vi "Scripting_ChangeBaseClassInSubClass.vi"(0 "SubClass":refnum<vi>, 1 "NewBaseClass":path=path "C:/Projects/Base2_class/Base2.lvclass", 2 "GOOP4Style":bool, 5 "error in (no error)":errorcluster) -> (19 "error out":errorcluster={"status"=TRUE, "code"=1055, "source"="Property Node in Scripting_ConvertBaseClassToSubClass.vi"})   [LabVIEW 2020]
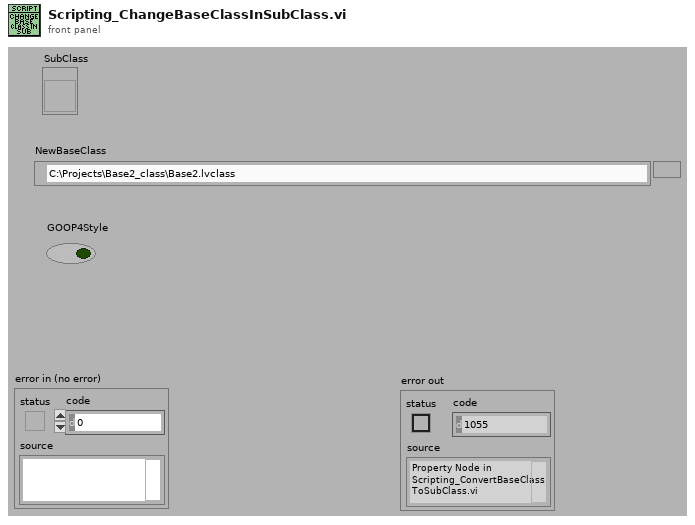
[diagram p1: front panel]
types:
  T1 = cluster{"NewBaseClass":refnum<vi>, "NewBaseClassPath":path, "SubClass":refnum<vi>, "NewBaseClassName":string, "AllBaseClassFiles":path[], "ClassVIs":refnum<vi>[], "CurrentBaseClassRef":refnum<vi>, "CurrentBaseClassPath":path, "CurrentRootBaseClassPath":path, "NewRootBaseClassPath":path}
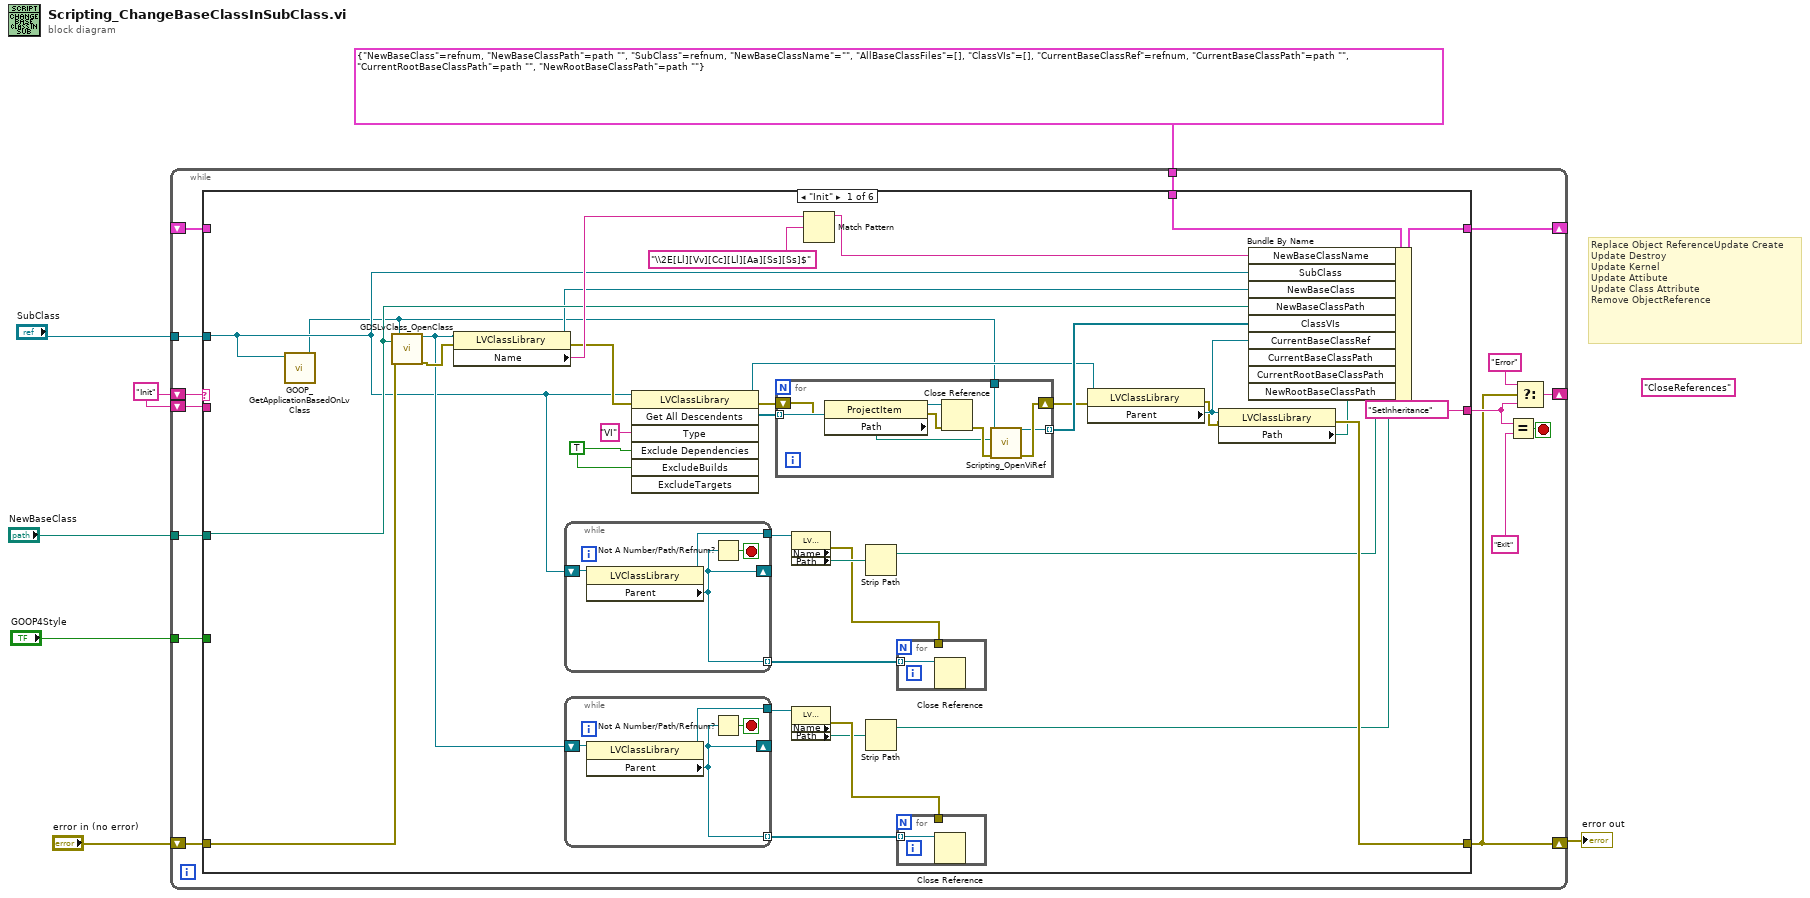
[diagram p0: block diagram]
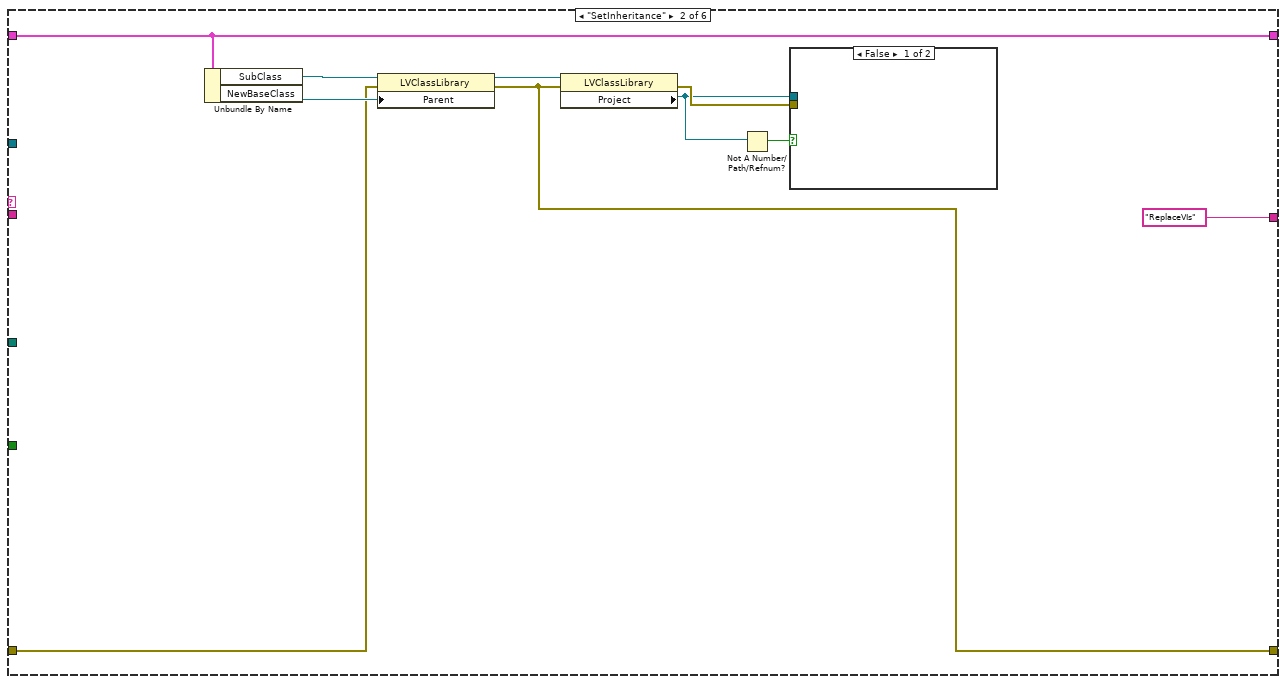
[diagram p2: hidden frame]
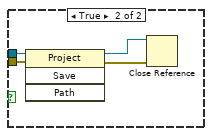
[diagram p3: hidden frame]
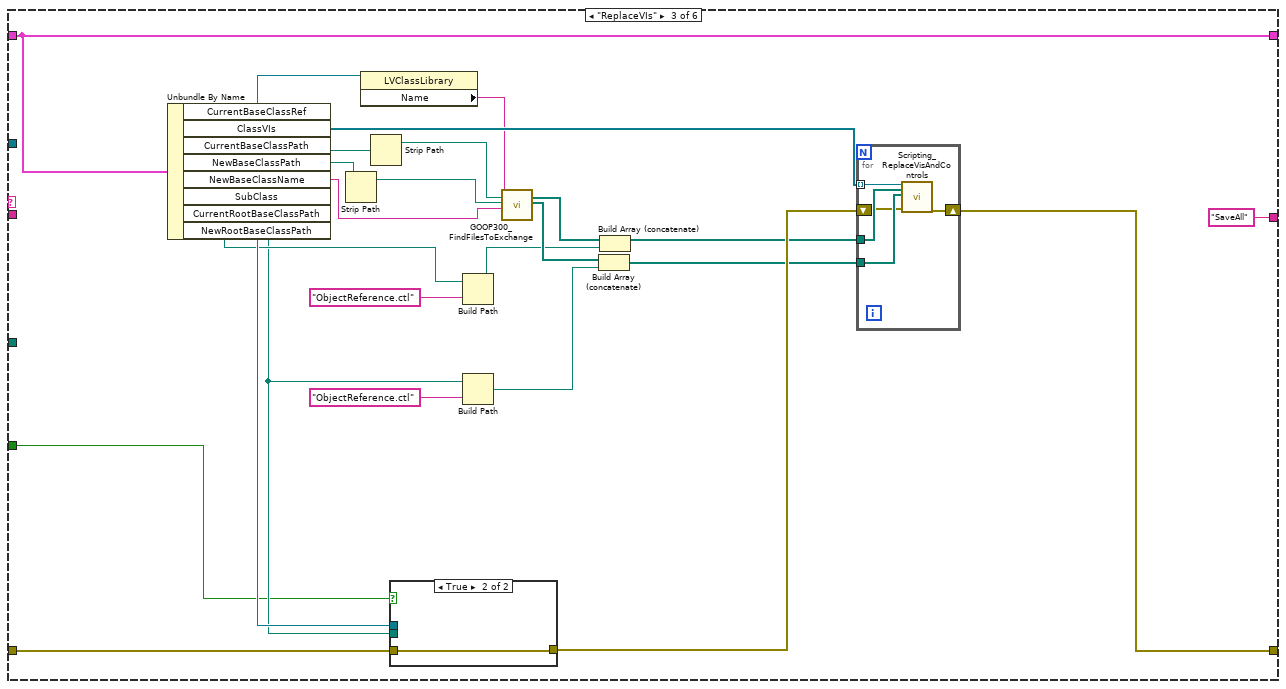
[diagram p4: hidden frame]
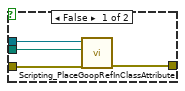
[diagram p5: hidden frame]
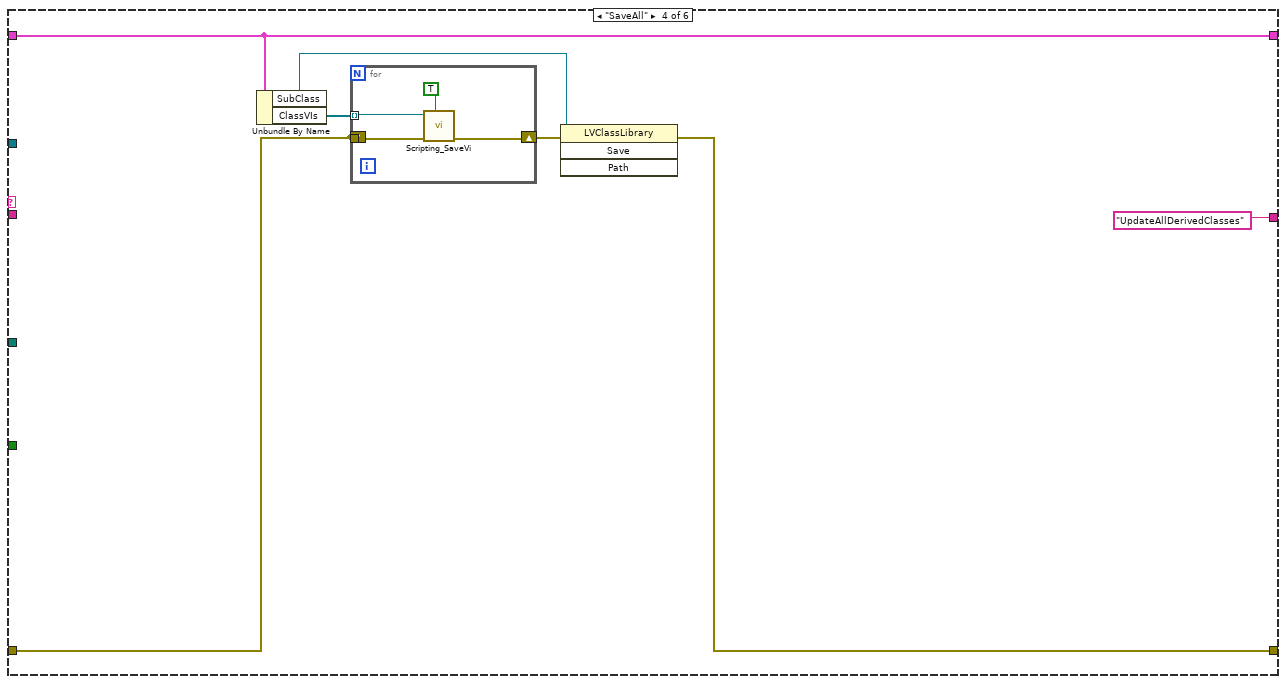
[diagram p6: hidden frame]
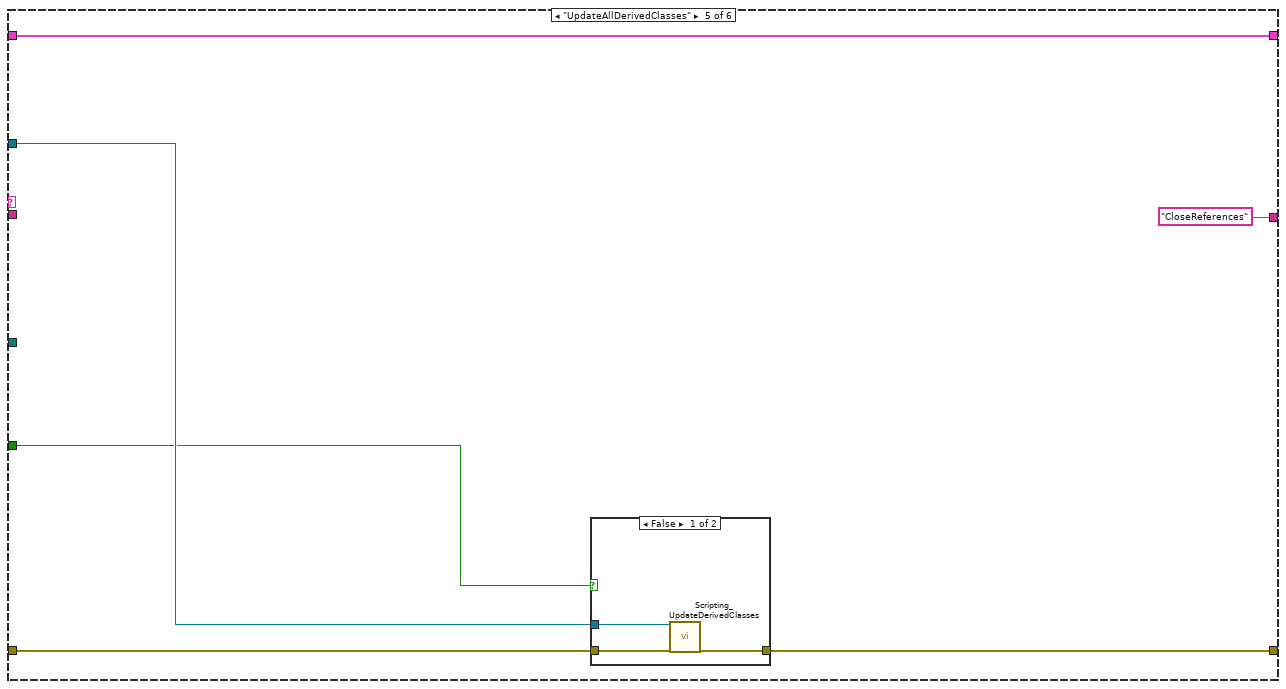
[diagram p7: hidden frame]
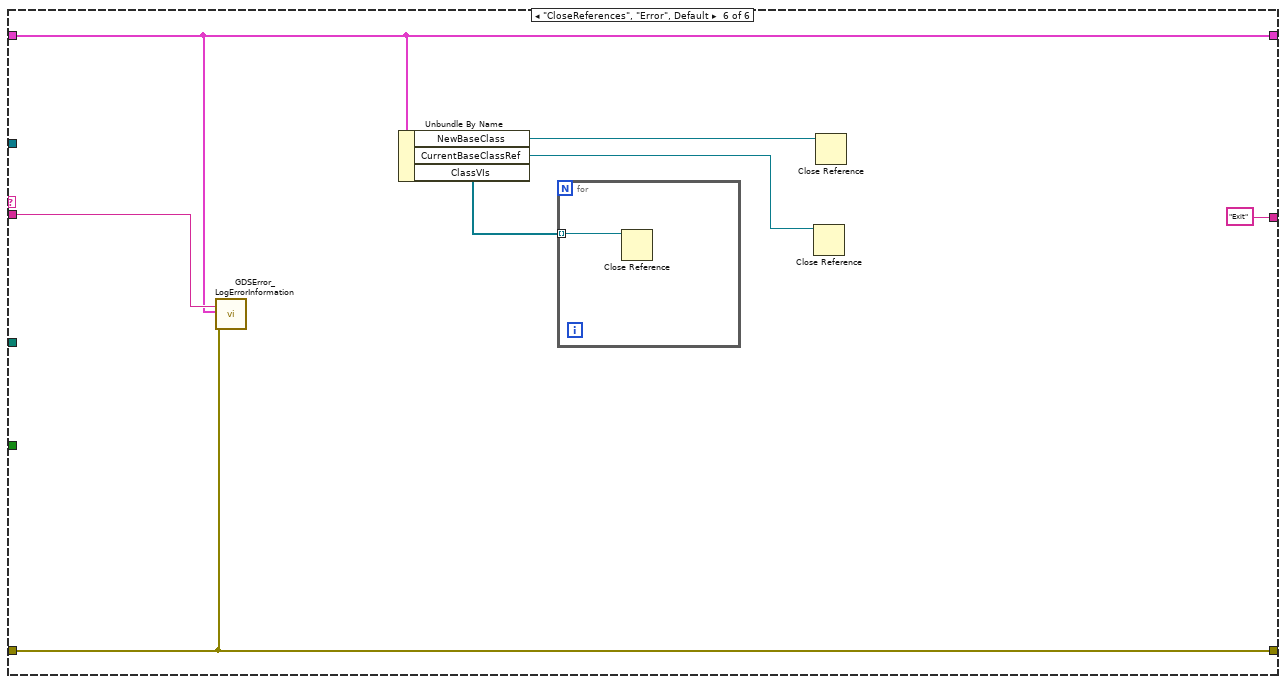
[diagram p9: hidden frame]
diagram:
  (unwired) "CloseReferences"
  w2 = "Init"
  # "Replace Object ReferenceUpdate Create\nUpdate Destroy\nUpdate Kernel\nUpdate Attibute\nUpdate Class Attribute\nRemove ObjectReference"
  n1 = while {
    shift-right: [w15] -> w6
    shift-left: "error in (no error)" -> [w22]
    shift-right: [w20] -> _
    shift-left: w2 -> [w21]
    shift-right: [w14] -> _
    shift-left: _ -> [w13]
    tunnel: "SubClass" -> [w12]
    tunnel: T1 {"NewBaseClass"=refnum, "NewBaseClassPath"=path "", "SubClass"=refnum, "NewBaseClassName"="", "AllBaseClassFiles"=[], "ClassVIs"=[], "CurrentBaseClassRef"=refnum, "CurrentBaseClassPath"=path "", "CurrentRootBaseClassPath"=path "", "NewRootBaseClassPath"=path ""} -> [w11]
    tunnel: "NewBaseClass" -> [w10]
    shift-left: w2 -> [w9]
    tunnel: "GOOP4Style" -> [w8]
    stop <- w19 stop-if-true
    n2 = case shown="\"Init\"" w21 {
      tunnel: w22 -> [w39 w83 w106 w130 w140 w149]
      tunnel: [w47 w77 w114 w127 w138 w149] -> w15
      tunnel: ["SetInheritance" "ReplaceVIs" "SaveAll" "UpdateAllDerivedClasses" "CloseReferences" "Exit"] -> w16
      tunnel: [w57 w85 w110 w131 w141 w147] -> w14
      tunnel: w13 -> [_ w85 w110 w131 w141 w147]
      tunnel: w12 -> [w24 _ _ _ w139 _]
      tunnel: w11 -> [w54 _ _ _ _ _]
      tunnel: w10 -> [w44 _ _ _ _ _]
      tunnel: w9 -> [_ _ _ _ _ w148]
      tunnel: w8 -> [_ _ w91 _ w137 _]
      frame "Init" {
        w25 = TRUE ("ExcludeDependencies")
        n3 = call "GOOP_GetApplicationBasedOnLvClass.vi"("LVClassLibrary in"=w24) -> ("Application out"=w23:refnum<vi>)  [unwired: 9 in, 1 out]
        n4 = call "GDSLvClass_OpenClass.vi"("ClassToOpen"=w44, "error in (no error)"=w39, "Project/ApplicationRef(If empty, currect active project will be used)"=w23) -> ("LVClass.Open"=w27:refnum<vi>, "error out"=w40:errorcluster)  [unwired: 15 in]
        n5 = property class="LVClassLibrary"(reference=w27, error in=w40) -> (reference out=w37:refnum<vi>, error out=w38:errorcluster, "Name"=w52:string)
        n6 = while {
          shift-right: [w65] -> _
          shift-left: w24 -> [w66]
          tunnel: [w65] -> w36 mode=indexing
          tunnel: [w64] -> w35
          stop <- w67 stop-if-true
          n7 = property class="LVClassLibrary"(reference=w66) -> (reference out=w64:refnum<vi>, "Parent"=w65:refnum<vi>)  [unwired: 1 in, 1 out]
          n8 = Not A Number/Path/Refnum?(number/path/refnum=w65) -> (NaN/Path/Refnum?=w67:bool)
        }
        n9 = while {
          shift-right: [w60] -> _
          shift-left: w27 -> [w61]
          tunnel: [w60] -> w28 mode=indexing
          tunnel: [w59] -> w29
          stop <- w62 stop-if-true
          n10 = property class="LVClassLibrary"(reference=w61) -> (reference out=w59:refnum<vi>, "Parent"=w60:refnum<vi>)  [unwired: 1 in, 1 out]
          n11 = Not A Number/Path/Refnum?(number/path/refnum=w60) -> (NaN/Path/Refnum?=w62:bool)
        }
        n12 = invoke class="LVClassLibrary" method="Get All Descendents"(reference=w24, error in=w38, "Type"="VI", "Exclude Dependencies"=w25, "ExcludeBuilds"=w25) -> (reference out=w43:refnum<vi>, error out=w55:errorcluster, "All Descendents"=w56:refnum<vi>[])  [unwired: 2 in, 4 out]
        n13 = for {
          tunnel: w56 -> [w76] mode=indexing
          shift-right: [w71] -> w48
          shift-left: w55 -> [w73]
          tunnel: [w69] -> w49 mode=indexing
          tunnel: w23 -> [w68]
          n14 = property class="ProjectItem"(reference=w76, error in=w73) -> (reference out=w75:refnum<vi>, error out=w74:errorcluster, "Path"=w70:path)
          n15 = Close Reference(reference=w75, error in (no error)=w74) -> (error out=w72:errorcluster)
          n16 = call "Scripting_OpenViRef.vi"("error in"=w72, "ViPath/ViName/Viref"=w70, "AppRef"=w68) -> ("error out"=w71:errorcluster, "vi reference"=w69:refnum<vi>)  [unwired: 6 in, 1 out]
        }
        n17 = property class="LVClassLibrary" props=["Name", "Path"](reference=w35) -> (error out=w33:errorcluster, "Path"=w34:path)  [unwired: 1 in, 2 out]
        n18 = property class="LVClassLibrary" props=["Name", "Path"](reference=w29) -> (error out=w31:errorcluster, "Path"=w30:path)  [unwired: 1 in, 2 out]
        n19 = Match Pattern(string=w52, regular expression="\\2E[Ll][Vv][Cc][Ll][Aa][Ss][Ss]$") -> (before substring=w51:string)  [unwired: 1 in, 3 out]
        n20 = Strip Path(path=w34) -> (stripped path=w32:path)  [unwired: 1 out]
        n21 = Strip Path(path=w30) -> (stripped path=w26:path)  [unwired: 1 out]
        n22 = for {
          tunnel: w36 -> [w63] mode=indexing
          tunnel: w33 -> [_]
          n23 = Close Reference(reference=w63) -> ()  [unwired: 1 in, 1 out]
        }
        n24 = for {
          tunnel: w28 -> [w58] mode=indexing
          tunnel: w31 -> [_]
          n25 = Close Reference(reference=w58) -> ()  [unwired: 1 in, 1 out]
        }
        n26 = property class="LVClassLibrary"(reference=w43, error in=w48) -> (error out=w42:errorcluster, "Parent"=w46:refnum<vi>)  [unwired: 1 out]
        n27 = property class="LVClassLibrary"(reference=w46, error in=w42) -> (error out=w47:errorcluster, "Path"=w45:path)  [unwired: 1 out]
        n28 = Bundle By Name(cluster=w54, "NewBaseClassName"=w51, "SubClass"=w24, "NewBaseClass"=w37, "NewBaseClassPath"=w44, "ClassVIs"=w49, "CurrentBaseClassRef"=w46, "CurrentBaseClassPath"=w45, "CurrentRootBaseClassPath"=w32, "NewRootBaseClassPath"=w26) -> (w57:T1)
      }
      frame "SetInheritance" {
        n29 = Unbundle By Name(w85) -> ("SubClass"=w86:refnum<vi>, "NewBaseClass"=w84:refnum<vi>)
        n30 = property class="LVClassLibrary"(reference=w86, error in=w83, "Parent"=w84) -> (reference out=w81:refnum<vi>, error out=w77:errorcluster)
        n31 = property class="LVClassLibrary"(reference=w81, error in=w77) -> (error out=w80:errorcluster, "Project"=w79:refnum<vi>)  [unwired: 1 out]
        n32 = Not A Number/Path/Refnum?(number/path/refnum=w79) -> (NaN/Path/Refnum?=w78:bool)
        n33 = case shown="False" w78 {
          tunnel: w80 -> [_ w88]
          tunnel: w79 -> [_ w87]
          frame False {
          }
          frame True {
            n34 = invoke class="Project" method="Save"(reference=w87, error in=w88) -> (reference out=w89:refnum<vi>, error out=w90:errorcluster)  [unwired: 2 in, 2 out]
            n35 = Close Reference(reference=w89, error in (no error)=w90) -> ()  [unwired: 1 out]
          }
        }
      }
      frame "ReplaceVIs" {
        n36 = Unbundle By Name(w110) -> ("CurrentBaseClassRef"=w94:refnum<vi>, "ClassVIs"=w109:refnum<vi>[], "CurrentBaseClassPath"=w113:path, "NewBaseClassPath"=w112:path, "NewBaseClassName"=w92:string, "SubClass"=w107:refnum<vi>, "CurrentRootBaseClassPath"=w99:path, "NewRootBaseClassPath"=w95:path)
        n37 = Strip Path(path=w112) -> (stripped path=w104:path)  [unwired: 1 out]
        n38 = property class="LVClassLibrary"(reference=w94) -> ("Name"=w93:string)  [unwired: 1 in, 2 out]
        n39 = Strip Path(path=w113) -> (stripped path=w108:path)  [unwired: 1 out]
        n40 = case shown="True" w91 {
          tunnel: w107 -> [w119 _]
          tunnel: w106 -> [w118 w120]
          tunnel: [w117 w120] -> w105
          tunnel: w95 -> [w116 _]
          frame False {
            n41 = call "Scripting_PlaceGoopRefInClassAttribute.vi"("error in"=w118, "ObjectRef_LvClassFolderPath"=w116, "ClassRefnum"=w119) -> ("error out"=w117:errorcluster)  [unwired: 1 in, 3 out]
          }
          frame True {
          }
        }
        n42 = Build Path(base path=w99, name or relative path="ObjectReference.ctl" ("element")) -> (appended path=w98:path)
        n43 = Build Path(base path=w95, name or relative path="ObjectReference.ctl" ("element")) -> (appended path=w96:path)
        n44 = call "GOOP300_FindFilesToExchange.vi"("OldClassName(Prefix or suffix for some VIs)"=w93, "OldFolderPath"=w108, "NewFolderPath"=w104, "NewClassName(Prefix or suffix for some VIs)"=w92) -> ("OldFiles"=w111:path[], "NewFileArray"=w102:path[])  [unwired: 14 in]
        n45 = Build Array (concatenate)(w102, w96) -> (w101:path[])
        n46 = Build Array (concatenate)(w111, w98) -> (w103:path[])
        n47 = for {
          shift-right: [w125] -> w114
          shift-left: w105 -> [w122]
          tunnel: w103 -> [w124]
          tunnel: w101 -> [w123]
          tunnel: w109 -> [w121] mode=indexing
          n48 = call "Scripting_ReplaceVisAndControls.vi"("ViRef"=w121, "OldVIsAndControls"=w124, "NewVIsAndControls"=w123, "error in (no error)"=w122) -> ("error out"=w125:errorcluster)  [unwired: 14 in, 1 out]
        }
      }
      frame "SaveAll" {
        n49 = Unbundle By Name(w131) -> ("SubClass"=w128:refnum<vi>, "ClassVIs"=w132:refnum<vi>[])
        n50 = for {
          tunnel: w132 -> [w136] mode=indexing
          shift-right: [w133] -> w129
          shift-left: w130 -> [_]
          tunnel: w130 -> [w134]
          n51 = call "Scripting_SaveVi.vi"("ForceResaving(False)"=TRUE, "error in (no error)"=w134, "VIRefToSaveIn"=w136) -> ("error out"=w133:errorcluster)  [unwired: 7 in, 1 out]
        }
        n52 = invoke class="LVClassLibrary" method="Save"(reference=w128, error in=w129) -> (error out=w127:errorcluster)  [unwired: 2 in, 3 out]
      }
      frame "UpdateAllDerivedClasses" {
        n53 = case shown="False" w137 {
          tunnel: w140 -> [w145 w146]
          tunnel: w139 -> [w144 _]
          tunnel: [w143 w146] -> w138
          frame False {
            n54 = call "Scripting_UpdateDerivedClasses.vi"("ClassRef"=w144, "error in (no error)"=w145) -> ("error out"=w143:errorcluster)  [unwired: 17 in]
          }
          frame True {
          }
        }
      }
      frame "CloseReferences", "Error", Default {
        n55 = call "GDSError_LogErrorInformation.vi"("State"=w148, "LocalVariableData"=w147, "error in (no error)"=w149) -> ()  [unwired: 16 in, 1 out]
        n56 = Unbundle By Name(w147) -> ("NewBaseClass"=w153:refnum<vi>, "CurrentBaseClassRef"=w151:refnum<vi>, "ClassVIs"=w150:refnum<vi>[])
        n57 = for {
          tunnel: w150 -> [w154] mode=indexing
          n58 = Close Reference(reference=w154) -> ()  [unwired: 1 in, 1 out]
        }
        n59 = Close Reference(reference=w151) -> ()  [unwired: 1 in, 1 out]
        n60 = Close Reference(reference=w153) -> ()  [unwired: 1 in, 1 out]
      }
    }
    n61 = Equal?(x=w16, y="Exit") -> (x = y?=w19:bool)
    n62 = Select(t="Error", s=w15, f=w16) -> (s? t:f=w20:string)
  }
  "error out" <- w6
